vi "VIH Utility - STR - Extract HTML or XML Section.vi"(8 "Contain (opt)":string, 9 "Section name":string="Item", 11 "HTML in":string) -> (1 "end":string, 2 "body":string, 3 "start":string, 4 "after":string, 5 "before":string)   [LabVIEW 2014]
doc: "::: VI Helpeks :::\nCopyright (c) 2000-2026 Konstantin Shifershteyn. All rights reserved."
panel:
  # "VI Helpeks\nCopyright (c) 2012-2026 Konstantin Shifershteyn"
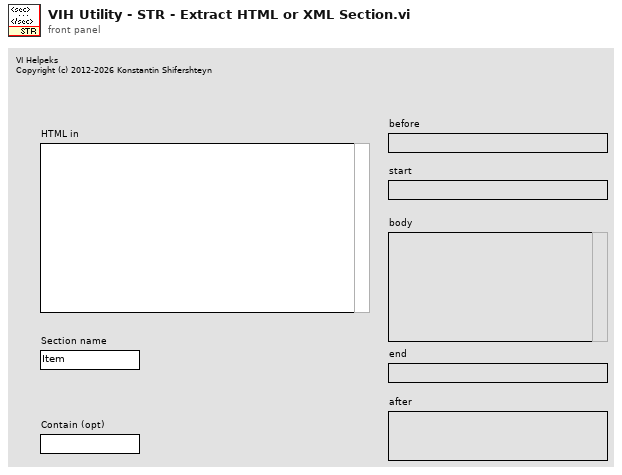
[diagram p1: front panel]
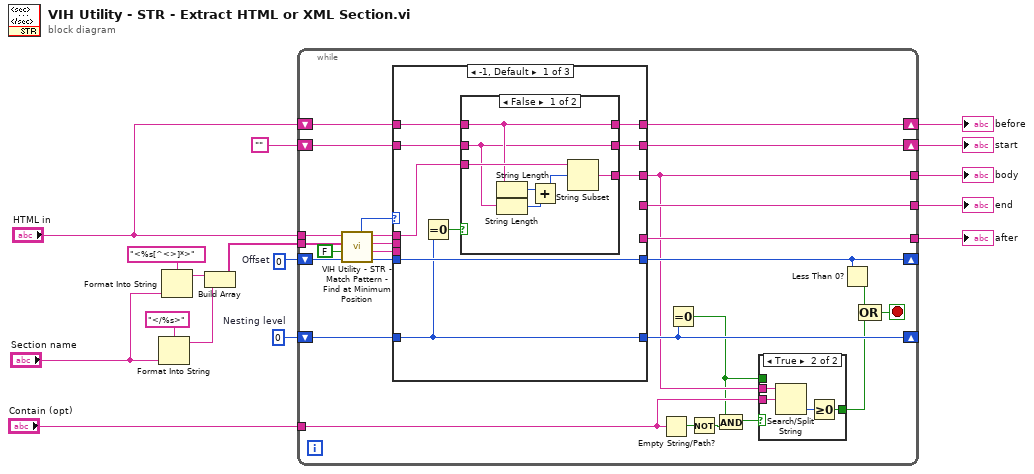
[diagram p0: block diagram]
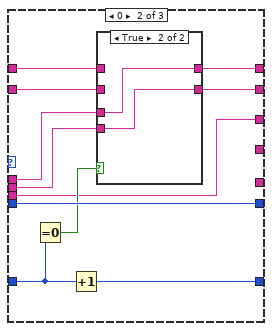
[diagram p4: hidden frame]
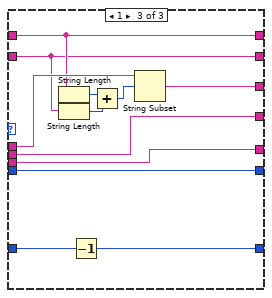
[diagram p6: hidden frame]
diagram:
  w2 = 0  # Nesting level
  w3 = 0  # Offset
  n1 = Format Into String(format string="</%s>" ("regular expression"), "Section name") -> (resulting string=w5:string)  [unwired: 2 in, 1 out]
  n2 = Format Into String(format string="<%s[^<>]*>" ("regular expression"), "Section name") -> (resulting string=w6:string)  [unwired: 2 in, 1 out]
  n3 = Build Array(w6, w5) -> (w4:string[])
  n4 = while {
    tunnel: "HTML in" -> [w43]
    tunnel: w4 -> [w42]
    shift-right: [w31] -> _
    shift-left: w3 -> [w41]
    shift-right: [w26] -> _
    shift-left: w2 -> [w38]
    shift-right: [w36] -> w11
    shift-left: "HTML in" -> [w37]
    shift-right: [w34] -> w13
    shift-left: "" -> [w35]
    tunnel: [w20] -> w15
    tunnel: [w30] -> w12
    tunnel: [w29] -> w10
    tunnel: "Contain (opt)" -> [w21]
    stop <- w25 stop-if-true
    n5 = call "VIH Utility - STR - Match Pattern - Find at Minimum Position.vi"("offset (0)"=w41, "case-sensitive (F)"=FALSE, "Regular expressions"=w42, "String"=w43) -> ("offset past match"=w39:i32, "after substring"=w28:string, "match substring"=w32:string, "before substring"=w33:string, "first match index"=w40:i32)  [unwired: 3 in]
    n6 = case shown="-1, Default" w40 {
      tunnel: [w57 w76 w91] -> w31
      tunnel: w39 -> [w57 w76 w91]
      tunnel: w38 -> [w56 w74 w92]
      tunnel: [w56 w75 w90] -> w26
      tunnel: w37 -> [w54 w72 w83]
      tunnel: [w53 w71 w83] -> w36
      tunnel: w35 -> [w51 w70 w82]
      tunnel: [w52 w69 w82] -> w34
      tunnel: w33 -> [w50 w68 w84]
      tunnel: w32 -> [_ w67 w89]
      tunnel: [w49 w66 w81] -> w20
      tunnel: [_ _ w89] -> w30
      tunnel: [_ _ w88] -> w29
      tunnel: w28 -> [_ w66 w88]
      frame -1, Default {
        n7 = Equal To 0?(x=w56) -> (x = 0?=w55:bool)
        n8 = case shown="False" w55 {
          tunnel: w54 -> [w59 _]
          tunnel: [w59 w65] -> w53
          tunnel: [w58 _] -> w52
          tunnel: w51 -> [w58 _]
          tunnel: w50 -> [w60 w65]
          tunnel: [w61 _] -> w49
          frame False {
            n9 = String Length(string=w59) -> (length=w63:i32)
            n10 = String Length(string=w58) -> (length=w62:i32)
            n11 = Add(x=w63, y=w62) -> (x+y=w64:i32)
            n12 = String Subset(string=w60, offset (0)=w64) -> (substring=w61:string)  [unwired: 1 in]
          }
          frame True {
          }
        }
      }
      frame 0 {
        n13 = Equal To 0?(x=w74) -> (x = 0?=w73:bool)
        n14 = Increment(x=w74) -> (x+1=w75:i32)
        n15 = case shown="True" w73 {
          tunnel: w72 -> [w78 _]
          tunnel: [w78 w80] -> w71
          tunnel: w70 -> [w77 _]
          tunnel: [w77 w79] -> w69
          tunnel: w68 -> [_ w80]
          tunnel: w67 -> [_ w79]
          frame False {
          }
          frame True {
          }
        }
      }
      frame 1 {
        n16 = String Length(string=w83) -> (length=w86:i32)
        n17 = String Length(string=w82) -> (length=w85:i32)
        n18 = Decrement(x=w92) -> (x-1=w90:i32)
        n19 = Add(x=w86, y=w85) -> (x+y=w87:i32)
        n20 = String Subset(string=w84, offset (0)=w87) -> (substring=w81:string)  [unwired: 1 in]
      }
    }
    n21 = Empty String/Path?(string/path=w21) -> (empty?=w24:bool)
    n22 = Equal To 0?(x=w26) -> (x = 0?=w18:bool)
    n23 = Not(x=w24) -> (.not. x?=w23:bool)
    n24 = And(x=w18, y=w23) -> (x .and. y?=w22:bool)
    n25 = case shown="True" w22 {
      tunnel: w21 -> [_ w48]
      tunnel: w20 -> [_ w47]
      tunnel: [w44 w45] -> w19
      tunnel: w18 -> [w44 _]
      frame False {
      }
      frame True {
        n26 = Search/Split String(string=w47, search string/char (-)=w48) -> (offset of match=w46:i32)  [unwired: 1 in, 2 out]
        n27 = Greater Or Equal To 0?(x=w46) -> (x >= 0?=w45:bool)
      }
    }
    n28 = Less Than 0?(x=w31) -> (x < 0?=w27:bool)
    n29 = Compound Arithmetic op=OR(w27, w19) -> (w25:bool)
  }
  "start" <- w13
  "end" <- w12
  "body" <- w15
  "before" <- w11
  "after" <- w10
